vi "MQTT Client - Configure TLS.vi"(0 "MQTT Session":T1, 1 "Trust OS trusted CAs?":bool=TRUE, 5 "Private Certificate (PEM)":path, 7 "Private Key (PEM)":path, 9 "Private Key Password (optional)":string, 11 "error in (no error)":errorcluster, 12 "Trusted Certificates (PEM)":path) -> (4 "MQTT Session out":T1, 15 "error out":errorcluster)   [LabVIEW 2019, in "KoRE-MQTT.lvlib"]
doc: "<b>Description:</b> This VI configures Transport Layer Security (TLS) settings for a MQTT client session. It establishes a secure connection utilizing the provided certificates and keys, ensuring that the MQTT broker is properly authenticated and that any server certificates not trusted by the operating system can be handled.\n\n<b>Input Terminals:</b>\n- <b>Trust OS trusted CAs? [1]</b>: Boolean value indicating whether to trust operating system trusted Certificate Authorities (CAs) by default.\n- <b>MQTT Session [0]</b>: Reference to the MQTT session that will utilize the configured TLS settings.\n- <b>Private Certificate (PEM) [5]</b>: The private certificate in PEM format used for client authentication with the broker; relevant only if the client needs to authenticate.\n- <b>Private Key [7]</b>: The private key corresponding to the private certificate, essential for establishing a secure connection when using client authentication.\n- <b>Private Key Password (optional) [9]</b>: Optional password for the private key, applicable if the private key is encrypted.\n- <b>Trusted Certificates (PEM) [12]</b>: Additional certificates in PEM format that can be trusted for the secure connection; relevant if server certificates are not trusted by the operating system.\n\n<b>Output Terminals:</b>\n- <b>MQTT Session out [4]</b>: Reference to the configured MQTT session with the applied TLS settings.\n\nNote: The MQTT broker hostname must be provided as a fully qualified domain name, as it will need to match the certificate for successful validation. Optional parameters are primarily needed if the user requires additional trust for server certificates or if client authentication is necessary, with the password being relevant only when the private key is encrypted.\n\n\nCopyright (c) 2025 KoRElibs.com\nSPDX-License-Identifier: EUPL-1.2\n\nThis VI is licensed under the European Union Public License (EUPL) Version 1.2. You may use this VI unmodified in proprietary works. If you distribute a modified version of this file, the modified file must be released under the EUPL-1.2. Full license: https://joinup.ec.europa.eu/asset/eupl/eupl/1.2/"
uses:
  KoRE-MQTT.lvlib
  TypeDefs/MQTT Client Session.ctl
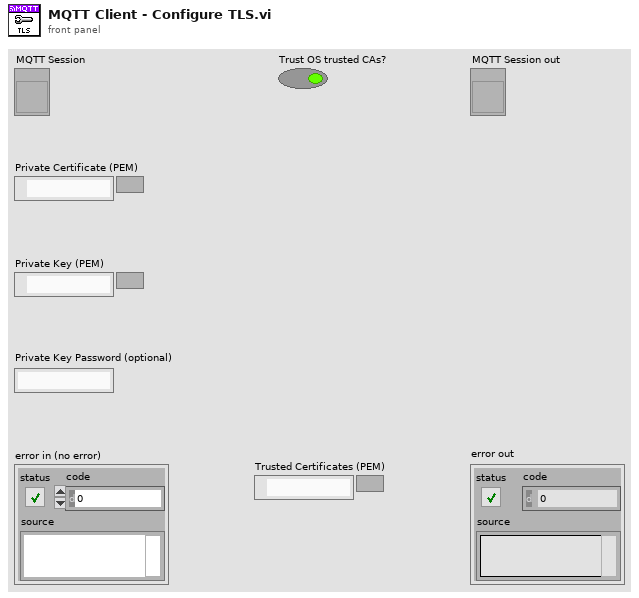
[diagram p1: front panel]
types:
  T1 = typedef "KoRE-MQTT.lvlib/MQTT Client Session.ctl" = refnum<vi>
  T2 = typedef "KoRE-MQTT.lvlib/MQTT Client Session - Data.ctl" = cluster{"TCP ref":refnum<k5>, "Next Packet Id":u16, "Version":u8, "Host":string, "Port":u16, "Ping Delta":u32, "Username":string, "Password":string, "Will QoS":u8, "Will Retain":bool, "Will Topic":string, "Will Payload":string, "TCP Timeout":i32, "Semaphore":T3, "In-Flight Messages":variant, "Close":bool, "Last Send":u32, "Keep Alive":u16, "Last Ping RTT":u32, "Last Ping":u32, "Will Properties":T4[], "Session Expiry Interval":u32, "Maximum QoS":u8, "Retain Available":bool, "Server Maximum Packet Size":u32, "Client Identifier":string, "Server Topic Alias Maximum":u16, "Wildcard Subscription Available":bool, "Subscription Identifier Available":bool, "Shared Subscription Available":bool, "Connect Properties":T5[], "Client Maximum Packet Size":u32, "Client Topic Alias Maximum":u16, "Server Receive Maximum":u16, "Client Receive Maximum":u16, "TLS cfg":refnum<k36>, "Subscriptions":T6[]}
  T3 = typedef "Semaphore RefNum" = refnum<k1>
  T4 = typedef "KoRE-MQTT.lvlib/MQTT Property - Will.ctl" = cluster{"Property":u8, "Value":string}
  T5 = typedef "KoRE-MQTT.lvlib/MQTT Property - CONNECT.ctl" = cluster{"Property":u8, "Value":string}
  T6 = typedef "KoRE-MQTT.lvlib/MQTT Subscription - Info.ctl" = cluster{"Packet Id":u16, "Index":u16, "Identifier":u32, "QoS":u8, "Topic Filter":string, "Reason Code":u8, "Reason String":string, "Granted":bool}
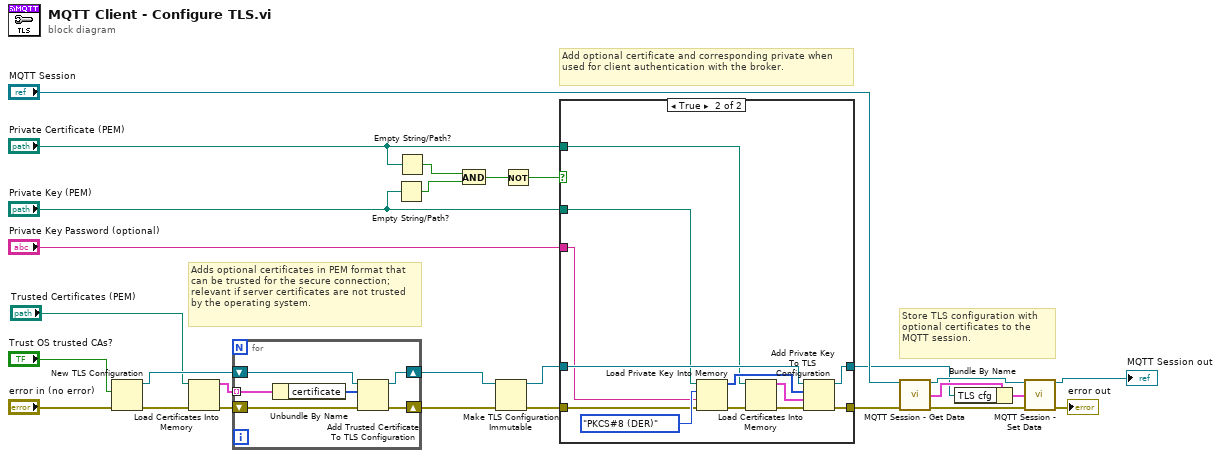
[diagram p0: block diagram]
diagram:
  # "Store TLS configuration with optional certificates to the MQTT session."
  # "Add optional certificate and corresponding private when used for client authentication with the broker."
  # "Adds optional certificates in PEM format that can be trusted for the secure connection; relevant if server certificates are not trusted by the operating system."
  n1 = New TLS Configuration(8:"error in (no error)", 10:"Trust OS trusted CAs?") -> (0:w23:errorcluster, 3:w22:refnum<k36>)
  n2 = Load Certificates Into Memory(8:w23, 11:"Trusted Certificates (PEM)") -> (0:w2:errorcluster, 3:w3:cluster{"certificate":u8[]}[])  [unwired: 1 in]
  n3 = for {
    tunnel: w3 -> [w33] mode=indexing
    shift-right: [w31] -> w20
    shift-left: w2 -> [w32]
    shift-right: [w28] -> w21
    shift-left: w22 -> [w29]
    n4 = Unbundle By Name(w33) -> ("certificate"=w30:u8[])
    n5 = Add Trusted Certificate To TLS Configuration(8:w32, 10:w30, 11:w29) -> (0:w31:errorcluster, 3:w28:refnum<k36>)
  }
  n6 = Empty String/Path?(string/path="Private Key (PEM)") -> (empty?=w4:bool)
  n7 = Empty String/Path?(string/path="Private Certificate (PEM)") -> (empty?=w5:bool)
  n8 = And(x=w5, y=w4) -> (x .and. y?=w7:bool)
  n9 = Make TLS Configuration Immutable(8:w20, 11:w21) -> (0:w9:errorcluster, 3:w17:refnum<k36>)
  n10 = Not(x=w7) -> (.not. x?=w6:bool)
  n11 = case shown="True" w6 {
    tunnel: w17 -> [w35 w47]
    tunnel: "Private Key (PEM)" -> [_ w45]
    tunnel: "Private Key Password (optional)" -> [_ w44]
    tunnel: [w35 w43] -> w11
    tunnel: "Private Certificate (PEM)" -> [_ w41]
    tunnel: w9 -> [w34 w39]
    tunnel: [w34 w36] -> w8
    frame False {
    }
    frame True {
      n12 = Load Private Key Into Memory(8:w39, 9:w44, 10:enum32{"PKCS#8 (PEM)", "PKCS#8 (DER)"}."PKCS#8 (DER)" ("format"), 11:w45) -> (0:w38:errorcluster, 3:w42:u8[])
      n13 = Load Certificates Into Memory(8:w38, 11:w41) -> (0:w37:errorcluster, 3:w40:cluster{"certificate":u8[]}[])  [unwired: 1 in]
      n14 = Add Private Key To TLS Configuration(8:w37, 9:w40, 10:w42, 11:w47) -> (0:w36:errorcluster, 3:w43:refnum<k36>)
    }
  }
  n15 = call "MQTT Session - Get Data.vi"("mqtt ref in"="MQTT Session", "error in"=w8) -> ("mqtt ref out"=w26:T1, "mqtt ref data"=w19:T2, "error out"=w14:errorcluster)  [unwired: 11 in]
  n16 = Bundle By Name(cluster=w19, "TLS cfg"=w11) -> (w18:T2)
  n17 = call "MQTT Session - Set Data.vi"("mqtt ref in"=w26, "mqtt ref data"=w18, "error in"=w14) -> ("mqtt ref out"=→"MQTT Session out":T1, "error out"=→"error out":errorcluster)  [unwired: 11 in]
